vi "Get Parameter Information.vi"(8 "error in":errorcluster, 11 "parameter value":variant) -> (0 "error out":errorcluster, 1 "repeated":bool, 2 "grpc type":T1, 3 "parameter name":string, 4 "message type":string)   [LabVIEW 2021, in "NI Measurement Plug-In SDK.lvlib"]
uses:
  NI Measurement Plug-In SDK.lvlib
  TypeDefs/Google Protobuf Field Kind.ctl
  <vilib>/Utility/Data Type/NI_Data Type.lvlib
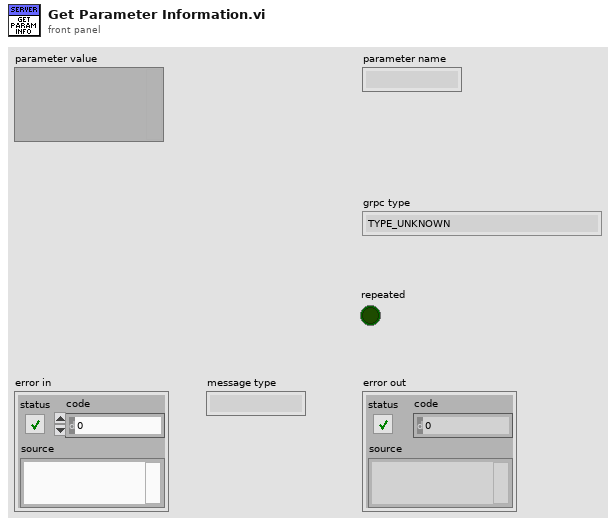
[diagram p1: front panel]
types:
  T1 = typedef "NI Measurement Plug-In SDK.lvlib/Google Protobuf Field Kind.ctl" = enum32{"TYPE_UNKNOWN", "TYPE_DOUBLE", "TYPE_FLOAT", "TYPE_INT64", "TYPE_UINT64", "TYPE_INT32", "TYPE_FIXED64", "TYPE_FIXED32", "TYPE_BOOL", "TYPE_STRING", "TYPE_GROUP", "TYPE_MESSAGE", "TYPE_BYTES", "TYPE_UINT32", "TYPE_ENUM", "TYPE_SFIXED32", "TYPE_SFIXED64", "TYPE_SINT32", "TYPE_SINT64"}
  T2 = typedef "NI_Data Type.lvlib/Data Type.ctl" = enum8{"Invalid Type", "Void", "I8", "I16", "I32", "I64", "U8", "U16", "U32", "U64", "Single Float", "Double Float", "Extended Float", "Single Complex", "Double Complex", "Extended Complex", "Enum U8", "Enum U16", "Enum U32", "Enum U64", "Single Float With Unit", "Double Float With Unit", "Extended Float With Unit", "Single Complex with Unit", "Double Complex with Unit", "Extended Complex with Unit", "Boolean", "String", "Path", "Picture", "Tag", "Array", "Cluster", "Variant", "LV Variant", "Waveform", "Timestamp", "Digital Waveform", "Digital Data", "ExpressData", "Refnum", "External Data", "VI", "Poly VI", "LabVIEW Class Instance", "Fixed Point", "Set Collection", "Map Collection"}
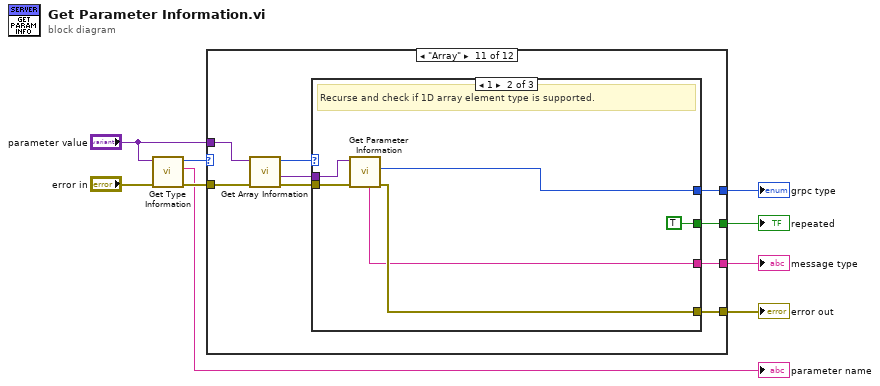
[diagram p0: block diagram]
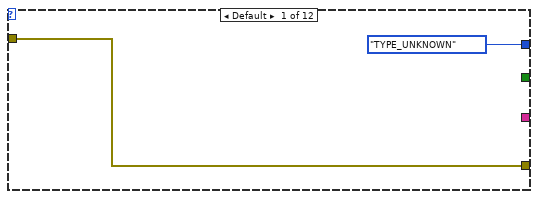
[diagram p2: hidden frame]
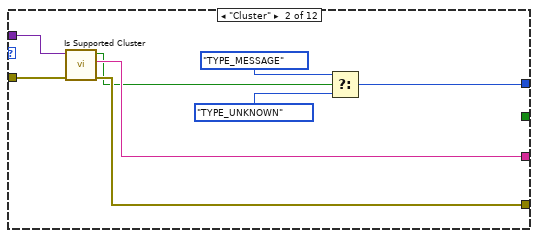
[diagram p3: hidden frame]
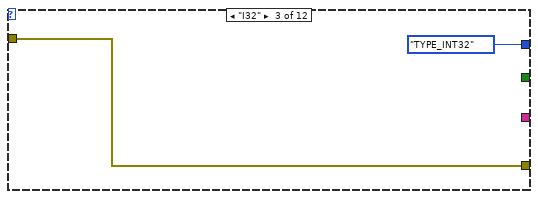
[diagram p4: hidden frame]
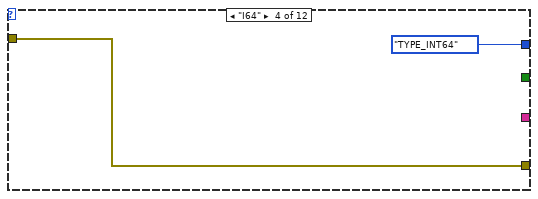
[diagram p5: hidden frame]
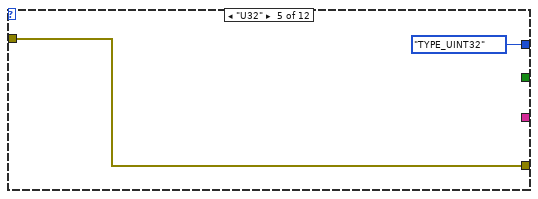
[diagram p6: hidden frame]
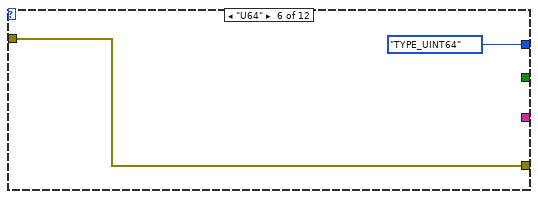
[diagram p7: hidden frame]
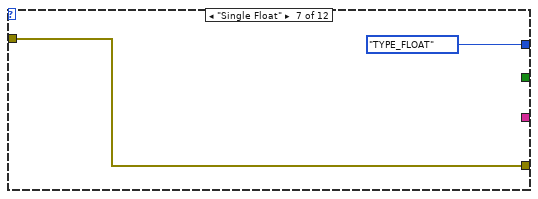
[diagram p8: hidden frame]
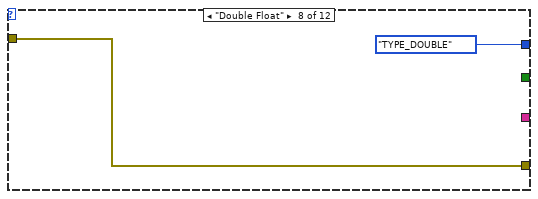
[diagram p9: hidden frame]
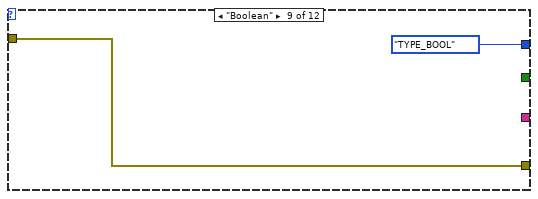
[diagram p10: hidden frame]
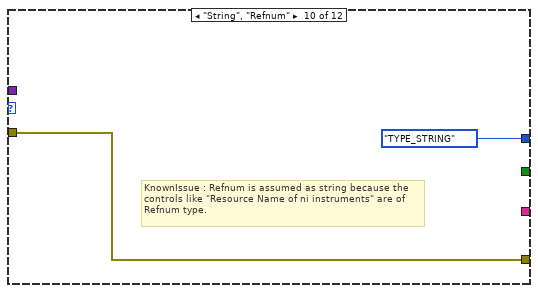
[diagram p11: hidden frame]
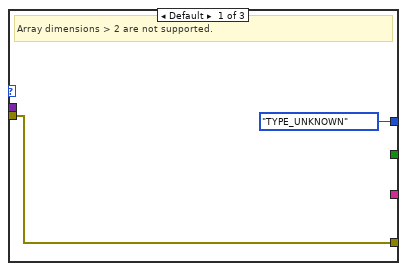
[diagram p12: hidden frame]
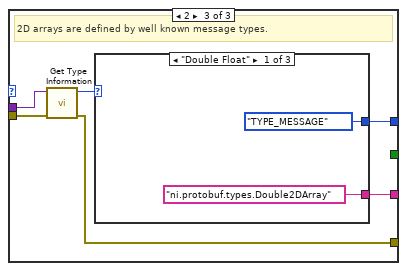
[diagram p13: hidden frame]
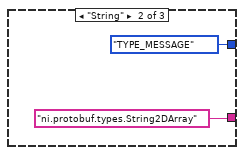
[diagram p14: hidden frame]
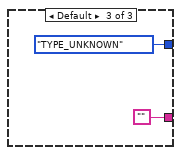
[diagram p15: hidden frame]
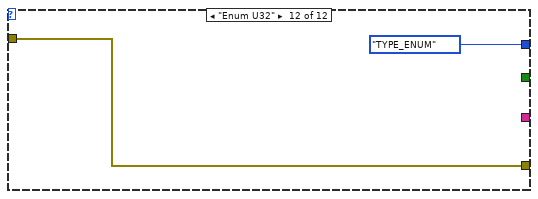
[diagram p16: hidden frame]
diagram:
  n1 = call <vilib>:"Get Type Information.vi"("error in (no error)"="error in", "variant"="parameter value") -> ("error out"=w8:errorcluster, "name"=→"parameter name":string, "type"=w9:T2)  [unwired: 5 in, 2 out]
  n2 = case shown="\"Array\"" w9 {
    tunnel: [Google_Protobuf_Field_Kind."TYPE_UNKNOWN" ("MessageElementType") w13 Google_Protobuf_Field_Kind."TYPE_INT32" ("MessageElementType") Google_Protobuf_Field_Kind."TYPE_INT64" ("MessageElementType") Google_Protobuf_Field_Kind."TYPE_UINT32" ("MessageElementType") Google_Protobuf_Field_Kind."TYPE_UINT64" ("MessageElementType") Google_Protobuf_Field_Kind."TYPE_FLOAT" ("MessageElementType") Google_Protobuf_Field_Kind."TYPE_DOUBLE" ("MessageElementType") Google_Protobuf_Field_Kind."TYPE_BOOL" ("MessageElementType") Google_Protobuf_Field_Kind."TYPE_STRING" ("MessageElementType") w39 Google_Protobuf_Field_Kind."TYPE_ENUM" ("MessageElementType")] -> w3
    tunnel: [_ _ _ _ _ _ _ _ _ _ w43 _] -> w4
    tunnel: w8 -> [w10 w18 w19 w21 w23 w25 w27 w29 w31 w33 w41 w65]
    tunnel: [w10 w18 w19 w21 w23 w25 w27 w29 w31 w33 w35 w65] -> w6
    tunnel: "parameter value" -> [_ w17 _ _ _ _ _ _ _ _ w42 _]
    tunnel: [_ w16 _ _ _ _ _ _ _ _ w38 _] -> w5
    frame Default {
    }
    frame "Cluster" {
      n3 = call "Is Supported Cluster.vi"("variant"=w17) -> ("message type"=w16:string, "supported?"=w12:bool)  [unwired: 9 in]
      n4 = Select(t=Google_Protobuf_Field_Kind."TYPE_MESSAGE" ("MessageElementType"), s=w12, f=Google_Protobuf_Field_Kind."TYPE_UNKNOWN" ("MessageElementType")) -> (s? t:f=w13:T1)
    }
    frame "I32" {
    }
    frame "I64" {
    }
    frame "U32" {
    }
    frame "U64" {
    }
    frame "Single Float" {
    }
    frame "Double Float" {
    }
    frame "Boolean" {
    }
    frame "String", "Refnum" {
      # "KnownIssue : Refnum is assumed as string because the controls like \"Resource Name of ni instruments\" are of Refnum type."
    }
    frame "Array" {
      n5 = call <vilib>:"Get Array Information.vi"("error in (no error)"=w41, "variant"=w42) -> ("error out"=w36:errorcluster, "array element data type"=w37:variant, "number of dimensions"=w40:i32)  [unwired: 6 in, 1 out]
      n6 = case shown="1" w40 {
        tunnel: [_ TRUE _] -> w43
        tunnel: [Google_Protobuf_Field_Kind."TYPE_UNKNOWN" ("MessageElementType") w49 w57] -> w39
        tunnel: [_ w48 w56] -> w38
        tunnel: w37 -> [_ w47 w55]
        tunnel: w36 -> [w44 w46 w54]
        tunnel: [w44 w50 w52] -> w35
        frame Default {
          # "Array dimensions > 2 are not supported."
        }
        frame 1 {
          # "Recurse and check if 1D array element type is supported."
          n7 = call "Get Parameter Information.vi"("error in"=w46, "parameter value"=w47) -> ("error out"=w50:errorcluster, "grpc type"=w49:T1, "message type"=w48:string)  [unwired: 5 in, 2 out]
        }
        frame 2 {
          # "2D arrays are defined by well known message types."
          n8 = call <vilib>:"Get Type Information.vi"("error in (no error)"=w54, "variant"=w55) -> ("error out"=w52:errorcluster, "type"=w53:T2)  [unwired: 5 in, 3 out]
          n9 = case shown="\"Double Float\"" w53 {
            tunnel: [Google_Protobuf_Field_Kind."TYPE_MESSAGE" ("MessageElementType") Google_Protobuf_Field_Kind."TYPE_MESSAGE" ("MessageElementType") Google_Protobuf_Field_Kind."TYPE_UNKNOWN" ("MessageElementType")] -> w57
            tunnel: ["ni.protobuf.types.Double2DArray" ("message_type") "ni.protobuf.types.String2DArray" ("message_type") ""] -> w56
            frame "Double Float" {
            }
            frame "String" {
            }
            frame Default {
            }
          }
        }
      }
    }
    frame "Enum U32" {
    }
  }
  "message type" <- w5
  "grpc type" <- w3
  "error out" <- w6
  "repeated" <- w4
